vi "Data Channel.vi"(8 "error in (no error)":errorcluster, 11 "Node Ptr":T6 format="%.0x") -> (0 "error out":errorcluster)   [LabVIEW 2020, in "Instrument Addon System Explorer.lvlib"]
uses:
  Instrument Addon System Explorer.lvlib
  <vilib>/NI VeriStand/Custom Device API/Custom Device API.lvlib
  Addon Shared/Instrument Addon Shared.lvlib
  Addon Shared/Types/FG Control.ctl
  <vilib>/NI VeriStand/Custom Device API/Custom Device Item Ref.ctl
  Addon Shared/Types/Protocol Data Type.ctl
  Addon Shared/Types/Data Channel Type.ctl
  Addon Shared/Types/Type Cast Type.ctl
  Addon Shared/Types/Endian.ctl
panel:
  in  "Delimiter":string=","
  in  "Reset":bool
  in  "Create":bool
  in  "Elements":u32
  in  "Units":string
  in  "Default Value":dbl
  in  "SHDocVw.IWebBrowser":refnum<k7>(container)
  out "Channel Type (Tab)":T1(tab)
  in  "Test Value":dbl
  in  "Format String":string="%.3g"
  out "Validated String":string
  in  "Expected String":string caption="Expected String (case sensitive)"
  in  "Endian":T2=enum."Little"
  in  "Type":T3
  in  "Enumerated List":i32(listbox)
  in  "Add":bool
  in  "Remove":bool
  in  "Channel Type":T4
  out "Data Type":T5
  in  "Header":cluster{"Section Name":string}={"Section Name"="Data Settings"}
  in  "Description":string
  in  "Name":string
  in  "Header 2":cluster{"Section Name":string}={"Section Name"="Data Format Settings"}
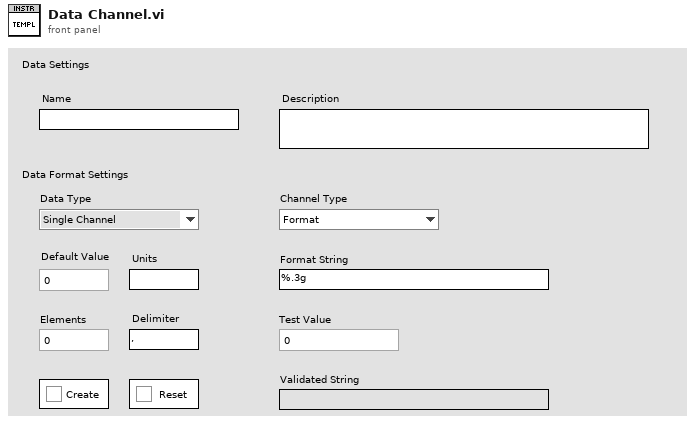
[diagram p1: front panel]
types:
  T1 = enum32{"Format", "Comparison", "Type Cast", "List"}
  T2 = typedef "Instrument Addon Shared.lvlib/Endian.ctl" = enum16{"Native", "Little", "Big"}
  T3 = typedef "Instrument Addon Shared.lvlib/Type Cast Type.ctl" = enum16{"DBL", "SGL", "U64", "U32", "U16", "U8", "I64", "I32", "I16", "I8"}
  T4 = typedef "Instrument Addon Shared.lvlib/Data Channel Type.ctl" = enum16{"Format", "Comparison", "Type Cast", "Enumerated List"}
  T5 = typedef "Instrument Addon Shared.lvlib/Protocol Data Type.ctl" = enum16{"Single Channel", "Array"}
  T6 = typedef "Custom Device API.lvlib/Custom Device Item Ref.ctl" = u64
  T7 = typedef "Instrument Addon Shared.lvlib/FG Control.ctl" = enum16{"Get", "Set"}
  T8 = typedef "Custom Device API.lvlib/Custom Device Item Info.ctl" = cluster{"Name":string, "Is Channel":bool, "GUID":string, "Is Waveform":bool}
  T9 = typedef "Instrument Addon Shared.lvlib/Data Parameters.ctl" = cluster{"Data Type":T5, "Channel Type":T4, "Format String":string, "Expected String":string, "Type":T3, "List":string[], "Delimiter":string, "Endian":T2}
  T10 = typedef "Custom Device API.lvlib/Custom Device Channel.ctl" = cluster{"Type":T11, "Units":string, "Default Value":dbl, "Faultable":bool, "Scalable":bool}
  T11 = typedef "Custom Device API.lvlib/Custom Device Channel Type.ctl" = enum16{"Input", "Output"}
  T12 = typedef "Custom Device API.lvlib/Custom Device Commands.ctl" = enum16{"Default", "Item renamed", "Shutdown", "Dynamic button pressed"}
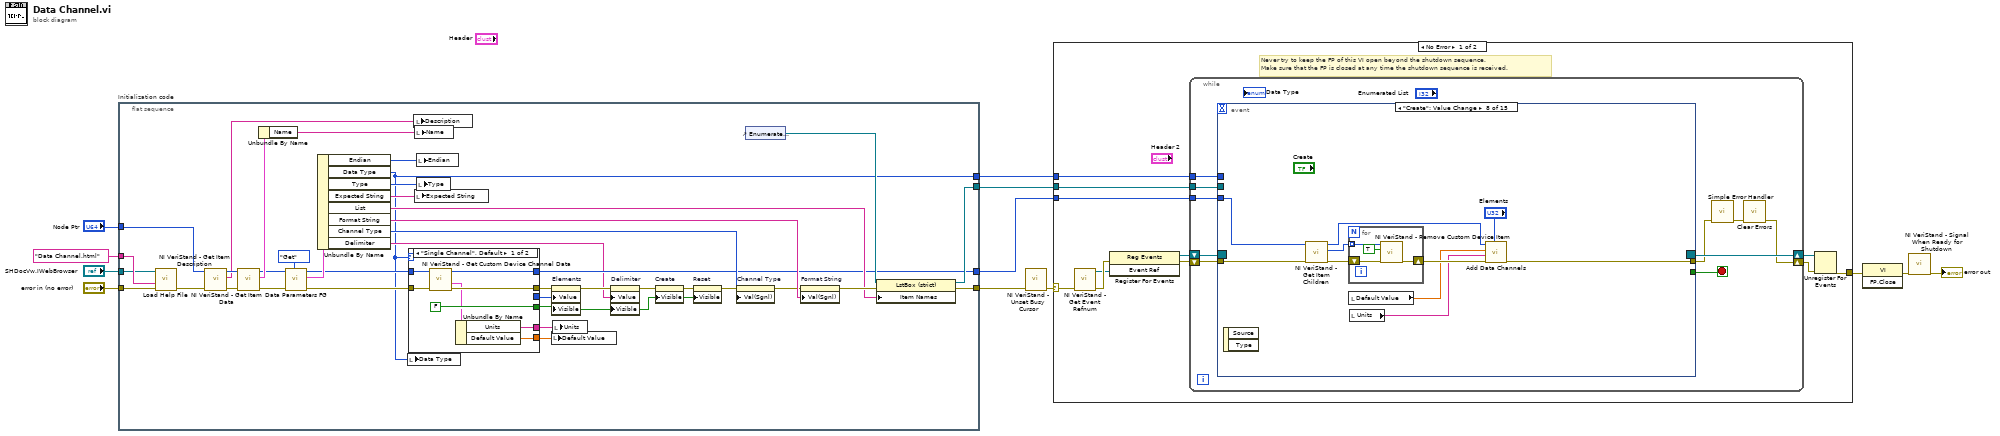
[diagram p0: block diagram]
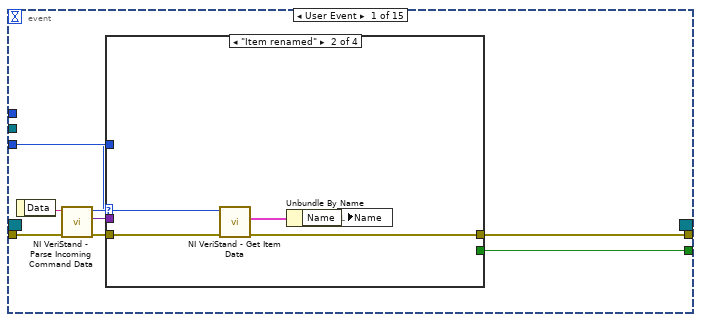
[diagram p2: hidden frame]
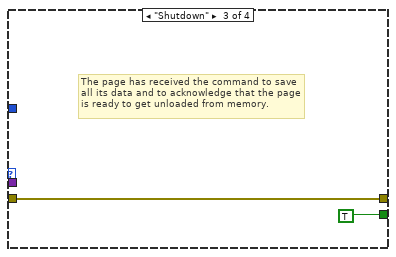
[diagram p4: hidden frame]
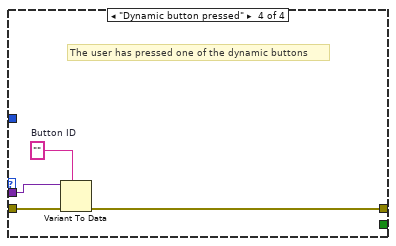
[diagram p5: hidden frame]
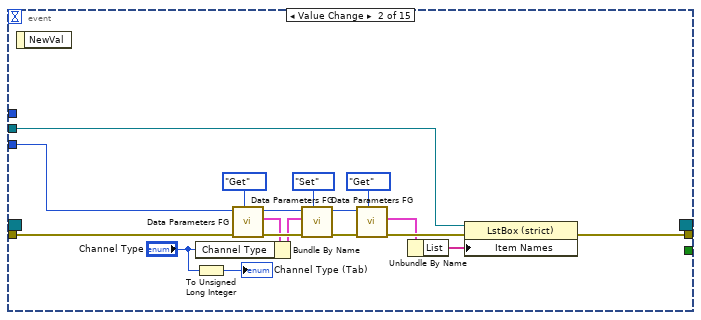
[diagram p6: hidden frame]
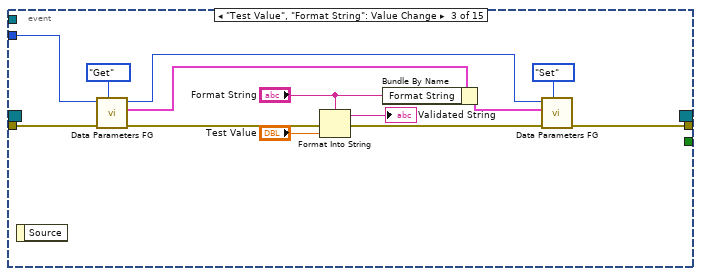
[diagram p7: hidden frame]
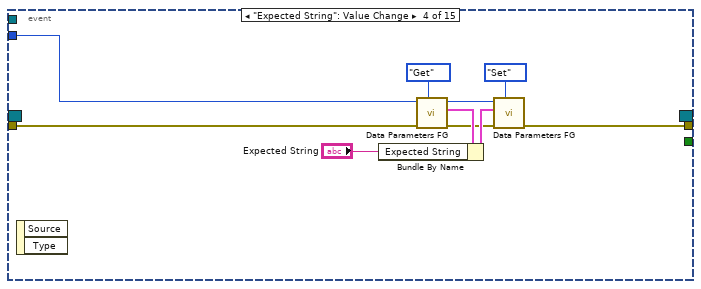
[diagram p8: hidden frame]
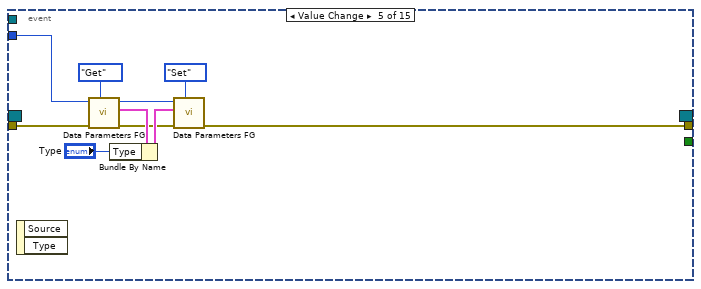
[diagram p9: hidden frame]
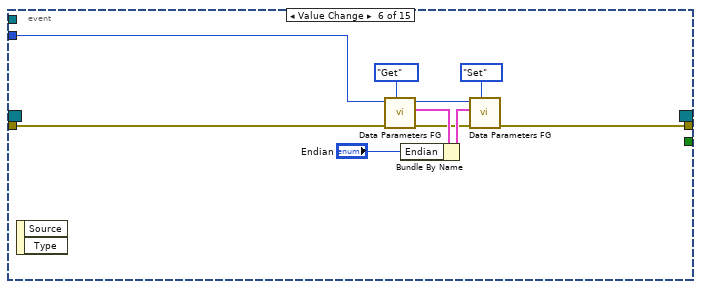
[diagram p10: hidden frame]
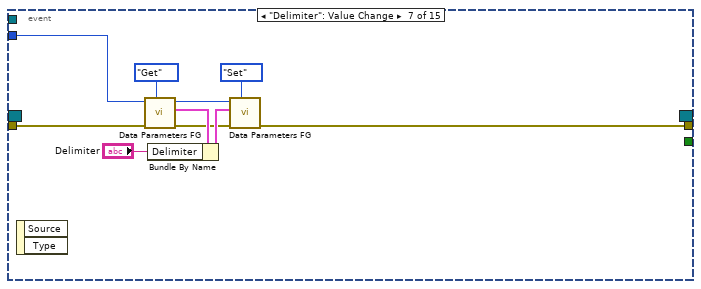
[diagram p11: hidden frame]
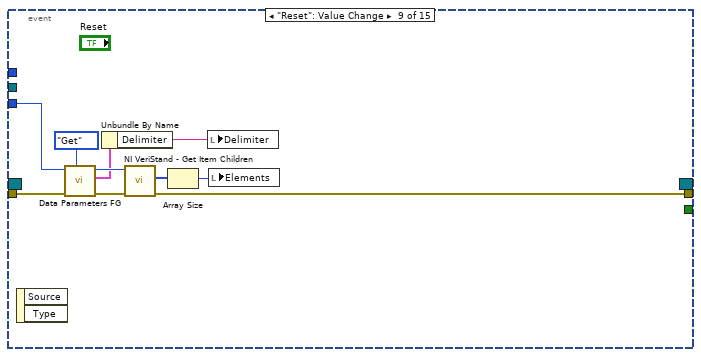
[diagram p12: hidden frame]
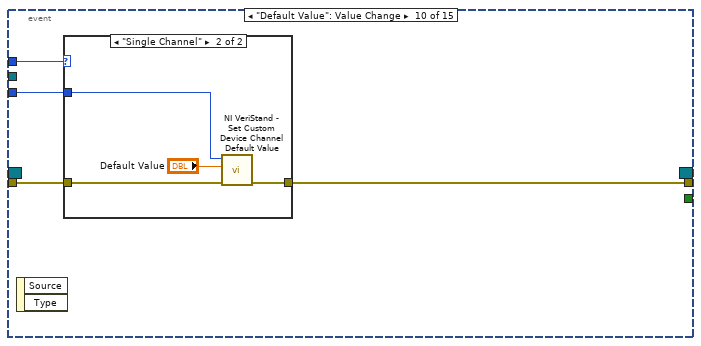
[diagram p13: hidden frame]
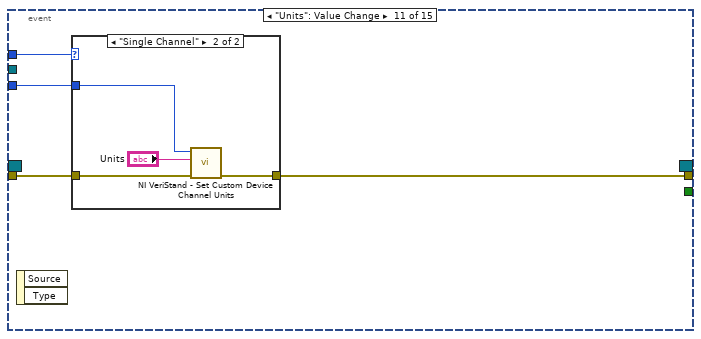
[diagram p15: hidden frame]
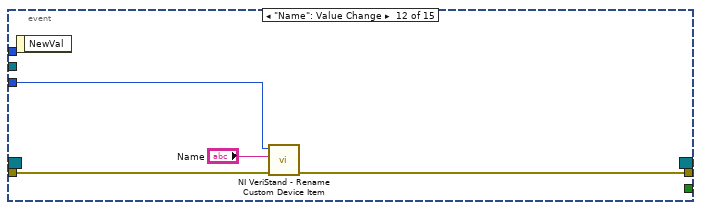
[diagram p17: hidden frame]
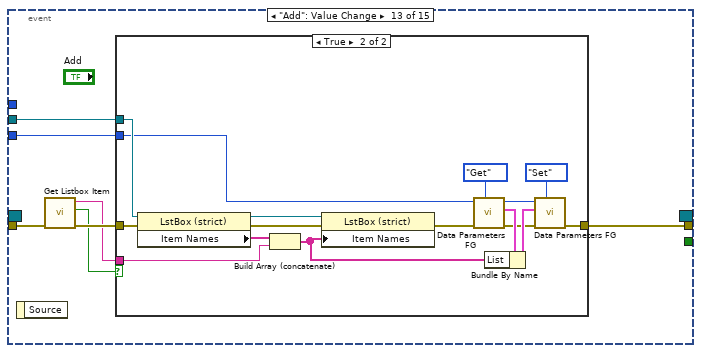
[diagram p18: hidden frame]
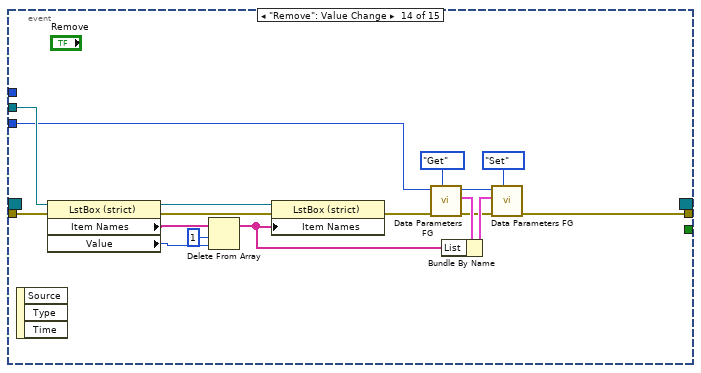
[diagram p20: hidden frame]
diagram:
  n1 = flat-sequence "Initialization code" {
    tunnel: "error in (no error)" -> [w45]
    tunnel: "Node Ptr" -> [w50]
    tunnel: [w33] -> w8
    tunnel: [w25] -> w5
    tunnel: "Data Channel.html" ("HTML File") -> [w43]
    tunnel: "SHDocVw.IWebBrowser" -> [w42]
    tunnel: [w30] -> w2
    tunnel: [w15] -> w1
    frame #0 {
      n2 = call "Load Help File.vi"("error in (no error)"=w45, "HTML File to Load"=w43, "SHDocVw.IWebBrowser2"=w42) -> ("error out"=w44:errorcluster)  [unwired: 8 in]
      n3 = call <vilib>:"NI VeriStand - Get Item Description.vi"("error in (no error)"=w44, "Item Ref in"=w50) -> ("error out"=w48:errorcluster, "Description"=w49:string, "Item Ref out"=w51:T6)  [unwired: 7 out]
      n4 = call <vilib>:"NI VeriStand - Get Item Data.vi"("error in (no error)"=w48, "Item Ref in"=w51) -> ("error out"=w29:errorcluster, "Item Info"=w47:T8, "Item Ref out"=w28:T6)  [unwired: 7 out]
      n5 = Unbundle By Name(w47) -> ("Name"=w46:string)
      n6 = call "Data Parameters FG.vi"("Action"=FG_Control."Get", "error in (no error)"=w29, "Item Ref in"=w28) -> ("error out"=w27:errorcluster, "Data Parameters"=w40:T9, "Item Ref out"=w26:T6)  [unwired: 6 in]
      n7 = Unbundle By Name(w40) -> ("Endian"=w14:T2, "Data Type"=w15:T5, "Type"=w35:T3, "Expected String"=w36:string, "List"=w31:string[], "Format String"=w39:string, "Channel Type"=w38:T4, "Delimiter"=w16:string)
      n8 = local write "Data Type"(w15) -> ()
      n9 = case shown="\"Single Channel\", Default" w15 {
        tunnel: [FALSE TRUE] -> w13
        tunnel: w27 -> [w58 w63]
        tunnel: w26 -> [w57 w67]
        tunnel: [w56 w62] -> w18
        tunnel: [w55 w64] -> w25
        tunnel: [w53 ""] -> w24
        tunnel: [w52 0.0 ("Default Value")] -> w23
        tunnel: [_ w60] -> w17
        frame "Single Channel", Default {
          n10 = call <vilib>:"NI VeriStand - Get Custom Device Channel Data.vi"("error in (no error)"=w58, "Channel Ref in"=w57) -> ("error out"=w56:errorcluster, "Channel"=w54:T10, "Channel Ref out"=w55:T6)  [unwired: 4 in, 3 out]
          n11 = Unbundle By Name(w54) -> ("Units"=w53:string, "Default Value"=w52:dbl)
        }
        frame "Array" {
          n12 = call <vilib>:"NI VeriStand - Get Item Children.vi"("error in (no error)"=w63, "Item Ref in"=w67) -> ("error out"=w62:errorcluster, "Child Refs"=w61:T6[], "Item Ref out"=w64:T6)  [unwired: 6 in, 1 out]
          n13 = Array Size(array=w61) -> (size(s)=w60:i32)
        }
      }
      n14 = local write "Description"(w49) -> ()
      n15 = local write "Name"(w46) -> ()
      n16 = local write "Expected String"(w36) -> ()
      n17 = local write "Endian"(w14) -> ()
      n18 = local write "Type"(w35) -> ()
      n19 = local write "Default Value"(w23) -> ()
      n20 = property on="Elements" class="DigNum (strict)"(error in=w18, "Value"=w17, "Visible"=w13) -> (error out=w22:errorcluster)  [unwired: 1 in, 1 out]
      n21 = local write "Units"(w24) -> ()
      n22 = property on="Delimiter" class="Str"(error in=w22, "Value"=w16, "Visible"=w13) -> (error out=w21:errorcluster)  [unwired: 1 in, 1 out]
      n23 = property on="Create" class="Bool"(error in=w21, "Visible"=w13) -> (error out=w20:errorcluster)  [unwired: 1 in, 1 out]
      n24 = property on="Reset" class="Bool"(error in=w20, "Visible"=w13) -> (error out=w19:errorcluster)  [unwired: 1 in, 1 out]
      n25 = property on="Channel Type" class="Enum (strict)"(error in=w19, "Val(Sgnl)"=w38) -> (error out=w37:errorcluster)  [unwired: 1 in, 1 out]
      n26 = control-ref of="Enumerated List"() -> (w32:refnum<vi>)
      n27 = property on="Format String" class="Str"(error in=w37, "Val(Sgnl)"=w39) -> (error out=w34:errorcluster)  [unwired: 1 in, 1 out]
      n28 = property class="LstBox (strict)"(reference=w32, error in=w34, "Item Names"=w31) -> (reference out=w30:refnum<vi>, error out=w33:errorcluster)
    }
  }
  n29 = call <vilib>:"NI VeriStand - Unset Busy Cursor.vi"("error in (no error)"=w8) -> ("error out"=w7:errorcluster)  [unwired: 10 out]
  n30 = case shown="No Error" w7 {
    selector: w7 -> [w71 w274]
    tunnel: [w76 w272] -> w12
    tunnel: w5 -> [w72 _]
    tunnel: w2 -> [w70 _]
    tunnel: w1 -> [w69 _]
    frame No Error {
      # "Never try to keep the FP of this VI open beyond the shutdown sequence.\nMake sure that the FP is closed at any time the shutdown sequence is received."
      n31 = call <vilib>:"NI VeriStand - Get Event Refnum.vi"("error in (no error)"=w71) -> ("error out"=w79:errorcluster, "Event Ref"=w75:refnum<user-event>)  [unwired: 9 out]
      n32 = register-events(error in=w79, w75) -> (reference out=w73:refnum<event-registration>, error out=w74:errorcluster)  [unwired: 1 in]
      n33 = while {
        tunnel: w72 -> [w85]
        shift-right: [w82] -> w77
        shift-left: w74 -> [w88]
        shift-right: [w89] -> w78
        shift-left: w73 -> [w87]
        tunnel: w70 -> [w81]
        tunnel: w69 -> [w80]
        stop <- w86 stop-if-true
        n34 = event shown="[7] \"Create\": Value Change" {
          selector: w87 -> [_ _ _ _ _ _ _ _ _ _ _ _ _ _ _]
          dyn-events: [_ _ _ _ _ _ _ _ _ _ _ _ _ _ _] -> w89
          timeout: _ -> [_ _ _ _ _ _ _ _ _ _ _ _ _ _ _]
          tunnel: w88 -> [w97 w121 w138 w148 w158 w168 w178 w187 w202 w208 w217 w226 w228 w253 w270]
          tunnel: [w93 _ _ _ _ _ _ _ _ _ _ _ _ _ _] -> w86
          tunnel: [w92 w110 w137 w147 w151 w167 w177 w185 w195 w207 w216 w225 w227 w254 w269] -> w84
          tunnel: w85 -> [w91 w119 w136 w146 w157 w166 w176 w186 w200 w206 w215 w224 w230 w251 w271]
          tunnel: w81 -> [_ w112 _ _ _ _ _ _ _ _ _ _ w229 w252 _]
          tunnel: w80 -> [_ _ _ _ _ _ _ _ _ w205 w214 _ _ _ _]
          event User Event {
            n35 = event-data() -> ("Data"=w96:string)  [unwired: 1 out]
            n36 = call <vilib>:"NI VeriStand - Parse Incoming Command Data.vi"("error in (no error)"=w97, "Incoming data"=w96) -> ("error out"=w95:errorcluster, "Outgoing data"=w90:variant, "Action"=w94:T12)  [unwired: 7 out]
            n37 = case shown="\"Item renamed\"" w94 {
              tunnel: w95 -> [w98 w103 w104 w109]
              tunnel: [_ _ TRUE _] -> w93
              tunnel: [w98 w100 w104 w106] -> w92
              tunnel: w91 -> [_ w102 _ _]
              tunnel: w90 -> [_ _ _ w108]
              frame "Default", Default {
              }
              frame "Item renamed" {
                n38 = call <vilib>:"NI VeriStand - Get Item Data.vi"("error in (no error)"=w103, "Item Ref in"=w102) -> ("error out"=w100:errorcluster, "Item Info"=w101:T8)  [unwired: 8 out]
                n39 = Unbundle By Name(w101) -> ("Name"=w99:string)
                n40 = local write "Name"(w99) -> ()
              }
              frame "Shutdown" {
                # "The page has received the command to save all its data and to acknowledge that the page is ready to get unloaded from memory."
              }
              frame "Dynamic button pressed" {
                w107 = ""  # Button ID
                # "The user has pressed one of the dynamic buttons"
                n41 = Variant To Data(error in=w109, type=w107, Variant=w108) -> (error out=w106:errorcluster)  [unwired: 1 out]
              }
            }
          }
          event Value Change {
            n42 = event-data() -> ()  [unwired: 2 out]
            n43 = To Unsigned Long Integer(number="Channel Type") -> (unsigned 32bit integer=→"Channel Type (Tab)":u32)
            n44 = call "Data Parameters FG.vi"("Action"=FG_Control."Get", "error in (no error)"=w121, "Item Ref in"=w119) -> ("error out"=w127:errorcluster, "Data Parameters"=w123:T9, "Item Ref out"=w125:T6)  [unwired: 6 in]
            n45 = Bundle By Name(cluster=w123, "Channel Type"="Channel Type") -> (w124:T9)
            n46 = call "Data Parameters FG.vi"("Action"=FG_Control."Set", "error in (no error)"=w127, "Data Parameters"=w124, "Item Ref in"=w125) -> ("error out"=w114:errorcluster, "Item Ref out"=w113:T6)  [unwired: 5 in, 1 out]
            n47 = call "Data Parameters FG.vi"("Action"=FG_Control."Get", "error in (no error)"=w114, "Item Ref in"=w113) -> ("error out"=w117:errorcluster, "Data Parameters"=w116:T9)  [unwired: 6 in, 1 out]
            n48 = Unbundle By Name(w116) -> ("List"=w115:string[])
            n49 = property class="LstBox (strict)"(reference=w112, error in=w117, "Item Names"=w115) -> (error out=w110:errorcluster)  [unwired: 1 out]
          }
          event "Test Value", "Format String": Value Change {
            n50 = event-data() -> ()  [unwired: 2 out]
            n51 = call "Data Parameters FG.vi"("Action"=FG_Control."Get", "error in (no error)"=w138, "Item Ref in"=w136) -> ("error out"=w132:errorcluster, "Data Parameters"=w128:T9, "Item Ref out"=w129:T6)  [unwired: 6 in]
            n52 = Format Into String(format string="Format String", error in=w132, "Test Value") -> (resulting string=→"Validated String":string, error out=w131:errorcluster)  [unwired: 1 in]
            n53 = Bundle By Name(cluster=w128, "Format String"="Format String") -> (w130:T9)
            n54 = call "Data Parameters FG.vi"("Action"=FG_Control."Set", "error in (no error)"=w131, "Data Parameters"=w130, "Item Ref in"=w129) -> ("error out"=w137:errorcluster)  [unwired: 5 in, 2 out]
          }
          event "Expected String": Value Change {
            n55 = event-data() -> ()  [unwired: 3 out]
            n56 = call "Data Parameters FG.vi"("Action"=FG_Control."Get", "error in (no error)"=w148, "Item Ref in"=w146) -> ("error out"=w141:errorcluster, "Data Parameters"=w143:T9, "Item Ref out"=w144:T6)  [unwired: 6 in]
            n57 = Bundle By Name(cluster=w143, "Expected String"="Expected String") -> (w145:T9)
            n58 = call "Data Parameters FG.vi"("Action"=FG_Control."Set", "error in (no error)"=w141, "Data Parameters"=w145, "Item Ref in"=w144) -> ("error out"=w147:errorcluster)  [unwired: 5 in, 2 out]
          }
          event Value Change {
            n59 = event-data() -> ()  [unwired: 3 out]
            n60 = call "Data Parameters FG.vi"("Action"=FG_Control."Get", "error in (no error)"=w158, "Item Ref in"=w157) -> ("error out"=w153:errorcluster, "Data Parameters"=w154:T9, "Item Ref out"=w155:T6)  [unwired: 6 in]
            n61 = Bundle By Name(cluster=w154, "Type"="Type") -> (w156:T9)
            n62 = call "Data Parameters FG.vi"("Action"=FG_Control."Set", "error in (no error)"=w153, "Data Parameters"=w156, "Item Ref in"=w155) -> ("error out"=w151:errorcluster)  [unwired: 5 in, 2 out]
          }
          event Value Change {
            n63 = event-data() -> ()  [unwired: 3 out]
            n64 = call "Data Parameters FG.vi"("Action"=FG_Control."Get", "error in (no error)"=w168, "Item Ref in"=w166) -> ("error out"=w162:errorcluster, "Data Parameters"=w163:T9, "Item Ref out"=w164:T6)  [unwired: 6 in]
            n65 = Bundle By Name(cluster=w163, "Endian"="Endian") -> (w165:T9)
            n66 = call "Data Parameters FG.vi"("Action"=FG_Control."Set", "error in (no error)"=w162, "Data Parameters"=w165, "Item Ref in"=w164) -> ("error out"=w167:errorcluster)  [unwired: 5 in, 2 out]
          }
          event "Delimiter": Value Change {
            n67 = event-data() -> ()  [unwired: 3 out]
            n68 = call "Data Parameters FG.vi"("Action"=FG_Control."Get", "error in (no error)"=w178, "Item Ref in"=w176) -> ("error out"=w172:errorcluster, "Data Parameters"=w173:T9, "Item Ref out"=w174:T6)  [unwired: 6 in]
            n69 = Bundle By Name(cluster=w173, "Delimiter"="Delimiter") -> (w175:T9)
            n70 = call "Data Parameters FG.vi"("Action"=FG_Control."Set", "error in (no error)"=w172, "Data Parameters"=w175, "Item Ref in"=w174) -> ("error out"=w177:errorcluster)  [unwired: 5 in, 2 out]
          }
          event "Create": Value Change {
            n71 = event-data() -> ()  [unwired: 3 out]
            n72 = call <vilib>:"NI VeriStand - Get Item Children.vi"("error in (no error)"=w187, "Item Ref in"=w186) -> ("error out"=w190:errorcluster, "Child Refs"=w189:T6[], "Item Ref out"=w183:T6)  [unwired: 6 in, 1 out]
            n73 = for {
              shift-right: [w193] -> w188
              shift-left: w190 -> [w191]
              tunnel: w189 -> [w192] mode=indexing
              n74 = call <vilib>:"NI VeriStand - Remove Custom Device Item.vi"("error in (no error)"=w191, "Force Delete (F)"=TRUE, "Item Ref in"=w192) -> ("error out"=w193:errorcluster)  [unwired: 7 in, 1 out]
            }
            n75 = local read "Default Value"() -> (w182:dbl)
            n76 = local read "Units"() -> (w181:string)
            n77 = call "Add Data Channels.vi"("# Elements"="Elements", "Error In"=w188, "Units"=w181, "Default Value"=w182, "Data Array Section Refnum In"=w183) -> ("Error Out"=w185:errorcluster)  [unwired: 6 in]
          }
          event "Reset": Value Change {
            n78 = event-data() -> ()  [unwired: 3 out]
            n79 = call "Data Parameters FG.vi"("Action"=FG_Control."Get", "error in (no error)"=w202, "Item Ref in"=w200) -> ("error out"=w201:errorcluster, "Data Parameters"=w198:T9, "Item Ref out"=w199:T6)  [unwired: 6 in]
            n80 = Unbundle By Name(w198) -> ("Delimiter"=w197:string)
            n81 = call <vilib>:"NI VeriStand - Get Item Children.vi"("error in (no error)"=w201, "Item Ref in"=w199) -> ("error out"=w195:errorcluster, "Child Refs"=w204:T6[])  [unwired: 6 in, 2 out]
            n82 = Array Size(array=w204) -> (size(s)=w196:i32)
            n83 = local write "Delimiter"(w197) -> ()
            n84 = local write "Elements"(w196) -> ()
          }
          event "Default Value": Value Change {
            n85 = event-data() -> ()  [unwired: 3 out]
            n86 = case shown="\"Single Channel\"" w205 {
              tunnel: w208 -> [w209 w213]
              tunnel: [w209 w212] -> w207
              tunnel: w206 -> [_ w211]
              frame "Array" {
              }
              frame "Single Channel" {
                n87 = call <vilib>:"NI VeriStand - Set Custom Device Channel Default Value.vi"("error in (no error)"=w213, "Default Value"="Default Value", "Channel Ref in"=w211) -> ("error out"=w212:errorcluster)  [unwired: 7 in, 1 out]
              }
            }
          }
          event "Units": Value Change {
            n88 = event-data() -> ()  [unwired: 3 out]
            n89 = case shown="\"Single Channel\"" w214 {
              tunnel: w217 -> [w218 w222]
              tunnel: [w218 w221] -> w216
              tunnel: w215 -> [_ w220]
              frame "Array" {
              }
              frame "Single Channel" {
                n90 = call <vilib>:"NI VeriStand - Set Custom Device Channel Units.vi"("error in (no error)"=w222, "Units"="Units", "Channel Ref in"=w220) -> ("error out"=w221:errorcluster)  [unwired: 7 in, 1 out]
              }
            }
          }
          event "Name": Value Change {
            n91 = event-data() -> ()  [unwired: 2 out]
            n92 = call <vilib>:"NI VeriStand - Rename Custom Device Item.vi"("error in (no error)"=w226, "New Name"="Name", "Item Ref in"=w224) -> ("error out"=w225:errorcluster)  [unwired: 1 in, 7 out]
          }
          event "Add": Value Change {
            n93 = event-data() -> ()  [unwired: 2 out]
            n94 = call "Get Listbox Item.vi"("error in (no error)"=w228) -> ("error out"=w233:errorcluster, "OK?"=w232:bool, "Item out"=w231:string)  [unwired: 8 in]
            n95 = case shown="True" w232 {
              tunnel: w229 -> [_ w250]
              tunnel: w233 -> [w234 w249]
              tunnel: w231 -> [_ w245]
              tunnel: [w234 w236] -> w227
              tunnel: w230 -> [_ w238]
              frame False {
              }
              frame True {
                n96 = property class="LstBox (strict)"(reference=w250, error in=w249) -> (reference out=w248:refnum<vi>, error out=w247:errorcluster, "Item Names"=w246:string[])
                n97 = Build Array (concatenate)(w246, w245) -> (w235:string[])
                n98 = property class="LstBox (strict)"(reference=w248, error in=w247, "Item Names"=w235) -> (error out=w237:errorcluster)  [unwired: 1 out]
                n99 = call "Data Parameters FG.vi"("Action"=FG_Control."Get", "error in (no error)"=w237, "Item Ref in"=w238) -> ("error out"=w239:errorcluster, "Data Parameters"=w243:T9, "Item Ref out"=w241:T6)  [unwired: 6 in]
                n100 = Bundle By Name(cluster=w243, "List"=w235) -> (w242:T9)
                n101 = call "Data Parameters FG.vi"("Action"=FG_Control."Set", "error in (no error)"=w239, "Data Parameters"=w242, "Item Ref in"=w241) -> ("error out"=w236:errorcluster)  [unwired: 5 in, 2 out]
              }
            }
          }
          event "Remove": Value Change {
            n102 = event-data() -> ()  [unwired: 4 out]
            n103 = property class="LstBox (strict)"(reference=w252, error in=w253) -> (reference out=w263:refnum<vi>, error out=w264:errorcluster, "Item Names"=w265:string[], "Value"=w266:i32)
            n104 = Delete From Array(array=w265, length=1, index=w266) -> (array with subset deleted=w255:string[])  [unwired: 1 out]
            n105 = property class="LstBox (strict)"(reference=w263, error in=w264, "Item Names"=w255) -> (error out=w256:errorcluster)  [unwired: 1 out]
            n106 = call "Data Parameters FG.vi"("Action"=FG_Control."Get", "error in (no error)"=w256, "Item Ref in"=w251) -> ("error out"=w257:errorcluster, "Data Parameters"=w261:T9, "Item Ref out"=w259:T6)  [unwired: 6 in]
            n107 = Bundle By Name(cluster=w261, "List"=w255) -> (w260:T9)
            n108 = call "Data Parameters FG.vi"("Action"=FG_Control."Set", "error in (no error)"=w257, "Data Parameters"=w260, "Item Ref in"=w259) -> ("error out"=w254:errorcluster)  [unwired: 5 in, 2 out]
          }
          event "Description": Value Change {
            n109 = event-data() -> ()  [unwired: 2 out]
            n110 = call <vilib>:"NI VeriStand - Set Item Description.vi"("error in (no error)"=w270, "Description"="Description", "Item Ref in"=w271) -> ("error out"=w269:errorcluster)  [unwired: 8 out]
          }
        }
        n111 = call <vilib>:"Simple Error Handler.vi"("error in (no error)"=w84) -> ("error out"=w83:errorcluster)  [unwired: 1 in, 7 out]
        n112 = call <vilib>:"Clear Errors.vi"("error in (no error)"=w83) -> ("error out"=w82:errorcluster)  [unwired: 1 in, 5 out]
      }
      n113 = Unregister For Events(event registration refnum=w78, error in=w77) -> (error out=w76:errorcluster)
    }
    frame Error {
      n114 = call <vilib>:"Simple Error Handler.vi"("error in (no error)"=w274) -> ("error out"=w273:errorcluster)  [unwired: 1 in, 7 out]
      n115 = call <vilib>:"Clear Errors.vi"("error in (no error)"=w273) -> ("error out"=w272:errorcluster)  [unwired: 1 in, 5 out]
    }
  }
  n116 = invoke class="VI" method="FP.Close"(error in=w12) -> (error out=w11:errorcluster)  [unwired: 2 in, 2 out]
  n117 = call <vilib>:"NI VeriStand - Signal When Ready for Shutdown.vi"("error in (no error)"=w11) -> ("error out"=→"error out":errorcluster)  [unwired: 10 out]
